vi "Check Writer Backpressure.vi"(8 "error in (no error)":errorcluster, 10 "Timeout (ms)":i32, 11 "CIF_CIPC_Chn in":refnum<class "CIF_Iceoryx_PCAP_Universal.lvclass">) -> (0 "error out":errorcluster, 2 "timed out?":bool)   [LabVIEW 2021, in "CIF_Iceoryx_PCAP_Universal.lvclass"]
uses:
  CIF_Iceoryx_PCAP_Universal.lvclass
  D:/dev/Packages/CIF_Channels_Core/src/CIFChannels/CIFChannels.lvclass
  CIFChannels/CIFChannels.lvclass/CIFChannels.ctl
  CIF_Iceoryx_PCAP_Universal.lvclass/CIF_Iceoryx_PCAP_Universal.ctl
  CIFChannels/Accessors/Read FIFO Backpressure.vi
  <vilib>/CIF Foundation/CIF Iceoryx/Iceoryx.lvlib
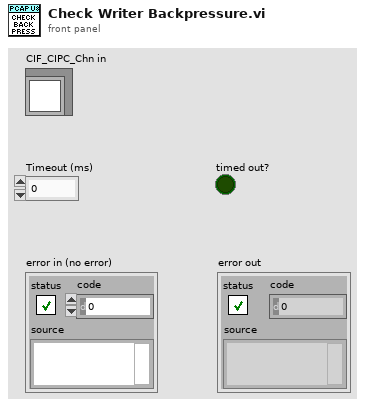
[diagram p1: front panel]
types:
  T1 = typedef "Iceoryx.lvlib/CIF Publisher Refnum.ctl" = cluster{"refnum":u64, "CIF Pub":enum8{"cifpub"}}
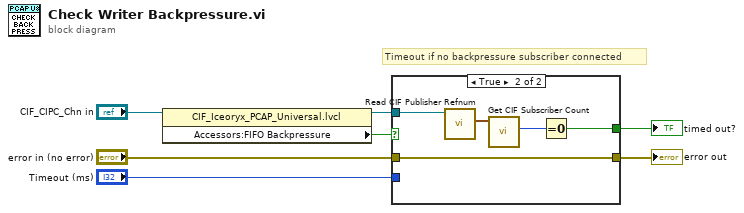
[diagram p0: block diagram]
diagram:
  # "Timeout if no backpressure subscriber connected"
  n1 = property class="CIF_Iceoryx_PCAP_Universal.lvcl"(reference="CIF_CIPC_Chn in") -> (reference out=w6:refnum<class "CIF_Iceoryx_PCAP_Universal.lvclass">, "Accessors:FIFO Backpressure"=w7:bool)  [unwired: 1 in, 1 out]
  n2 = case shown="True" w7 {
    tunnel: [w8 w11] -> w2
    tunnel: "error in (no error)" -> [w8 w11]
    tunnel: w6 -> [_ w12]
    tunnel: [_ w9] -> w1
    tunnel: "Timeout (ms)" -> [_ _]
    frame False {
    }
    frame True {
      n3 = call "Read CIF Publisher Refnum.vi"("CIF_Iceoryx_PCAP_Universal in"=w12) -> ("CIF Publisher Refnum"=w13:T1)  [unwired: 8 in, 2 out]
      n4 = call <vilib>:"Get CIF Subscriber Count.vi"("Publisher Reference"=w13) -> ("Backpressure"=w10:u32)  [unwired: 8 in, 2 out]
      n5 = Equal To 0?(x=w10) -> (x = 0?=w9:bool)
    }
  }
  "error out" <- w2
  "timed out?" <- w1
